vi "FlatToRichauth_ValidateTokenResponse.vi"(5 "OutputClusterType":T1, 11 "InputCluster":T2) -> (3 "OutputCluster":T1)   [LabVIEW 2020, in "grpc-auth_client.lvlib"]
uses:
  grpc-auth_client.lvlib
  auth_ValidateTokenResponse_Flat.ctl
  auth_ValidateTokenResponse.ctl
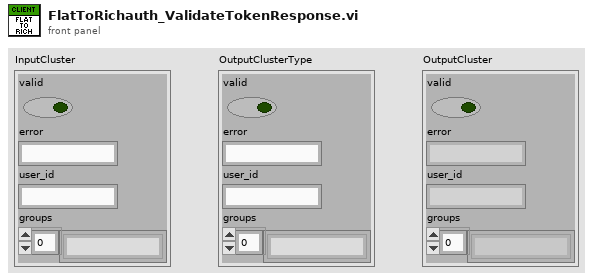
[diagram p1: front panel]
types:
  T1 = typedef "grpc-auth_client.lvlib/auth_ValidateTokenResponse.ctl" = cluster{"valid":bool, "error":string, "user_id":string, "groups":string[]}
  T2 = typedef "grpc-auth_client.lvlib/auth_ValidateTokenResponse_Flat.ctl" = cluster{"valid":bool, "error":string, "user_id":string, "groups":string[]}
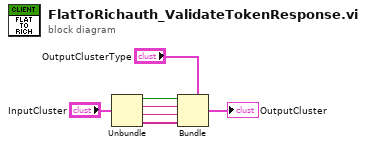
[diagram p0: block diagram]
diagram:
  n1 = Unbundle "Unbundle"("InputCluster") -> ("valid"=w4:bool, "error"=w3:string, "user_id"=w2:string, "groups"=w1:string[])
  n2 = Bundle "Bundle"(cluster="OutputClusterType", "valid"=w4, "error"=w3, "user_id"=w2, "groups"=w1) -> (→"OutputCluster":T1)
